vi "GAP_AcquireImagesV3_0.vi"() -> ()   [LabVIEW 2020]
uses:
  <vilib>/vision/driver/IMAQdx.llb/IMAQdx Buffer Number Mode.ctl
  <vilib>/vision/driver/NI_Vision_Acquisition_Software.lvlib
  <vilib>/vision/NI_Vision_Development_Module.lvlib
  <resource>/objmgr/imaqdx.rc
panel:
  out "Histogram":T1(graph)
  in  "Tab Control":enum32{"Acquisition"}(tab)
  in  "Camera Name":refnum<k21> caption="IMAQdx Session"
  out "Original Image":T2(plugin-control)
  out "Grayscale Image":T2(plugin-control)
  out "Acquired imgs":u32
  out "Frame rate":dbl
  in  "Overwrite Mode":u16(ring) items=["Get Oldest"=0, "Fail"=2, "Get Newest"=3]
  in  "Percent of Images Reserved by Driver":dbl=50.0
  out "Line profile data":T3 {"Minimum grayscale value" format="%.2f"; "Std. dev. of pixels values [ % ]" format="%.2f"; "Mean value of pixels values" format="%.2f"; "Maximum grayscale value" format="%.2f"}
  out "Line Profile":cluster{"x0":sgl, "dx":sgl, "Pixels Line":sgl[]}(graph)
  in  "Start acquisition":bool
  in  "Stop image acquisition":bool
  in  "Save image":bool
  in  "Stop program":bool
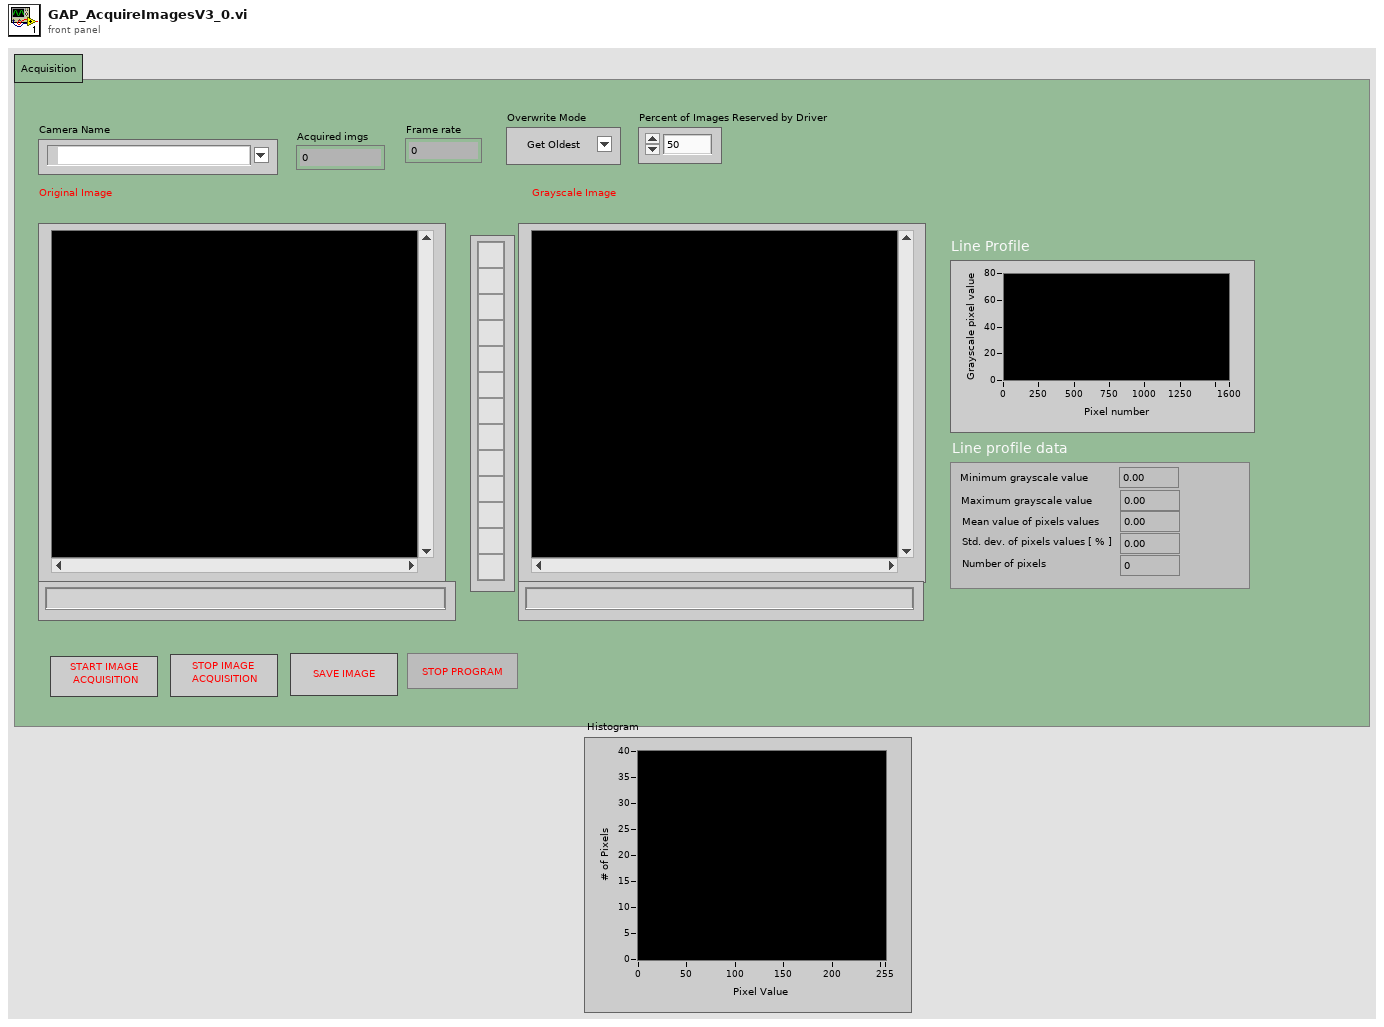
[diagram p1: front panel]
types:
  T1 = cluster{"Starting Value":sgl, "Incremental Value":sgl, "Histogram":u32[]}
  T2 = typedef "IMAQ Image.ctl" = refnum<image>
  T3 = cluster{"Minimum grayscale value":sgl, " Maximum grayscale value":sgl, "Mean value of pixels values":sgl, "Std. dev. of pixels values [ % ]":sgl, "Number of pixels":i32}
  T4 = typedef "NI_Vision_Acquisition_Software.lvlib/IMAQdx Buffer Number Mode.ctl" = enum32{"Next", "Last", "Buffer Number", "Every", "Last New"}
  T5 = typedef "Image Type" = u32
  T6 = typedef "IMAQdx.ctl" = refnum<k21>
  T7 = cluster{"Min":sgl, "Max":sgl, "Mean":sgl, "Std Dev":sgl, "Count":i32}
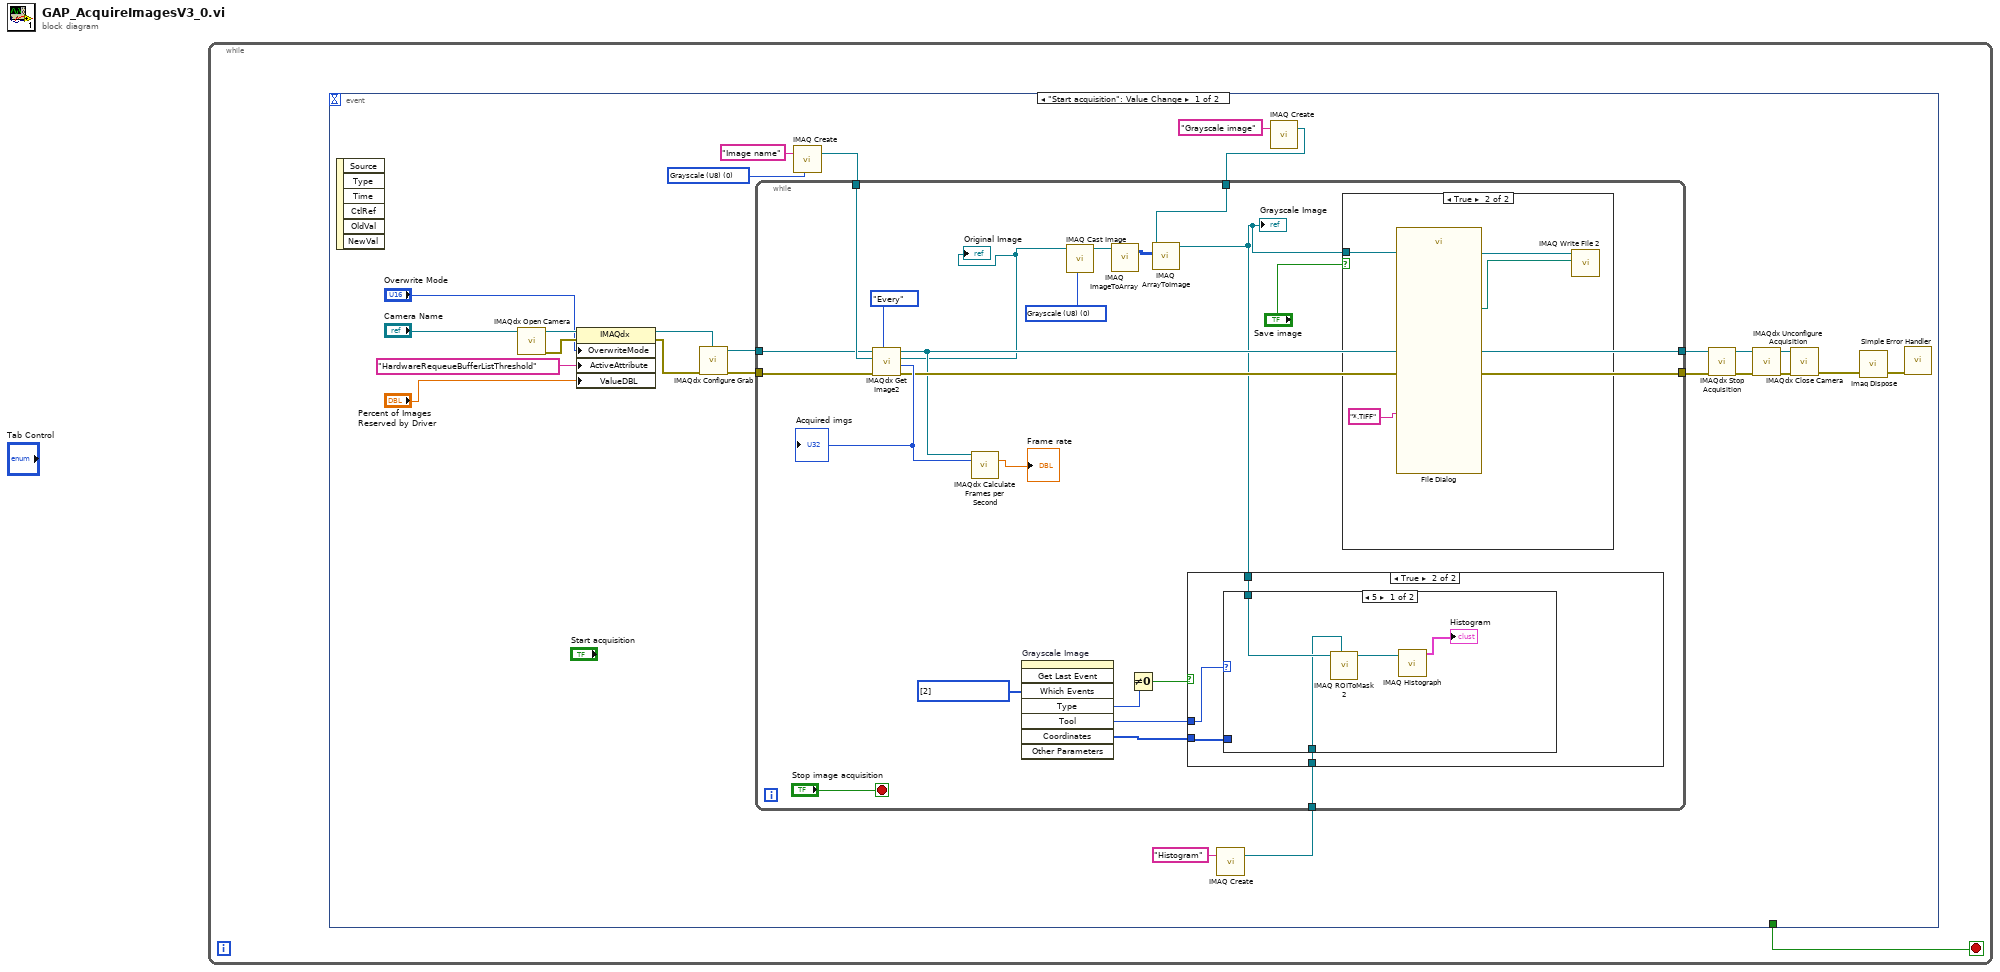
[diagram p0: block diagram]
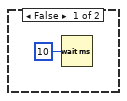
[diagram p3: hidden frame]
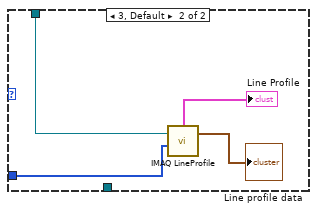
[diagram p4: hidden frame]
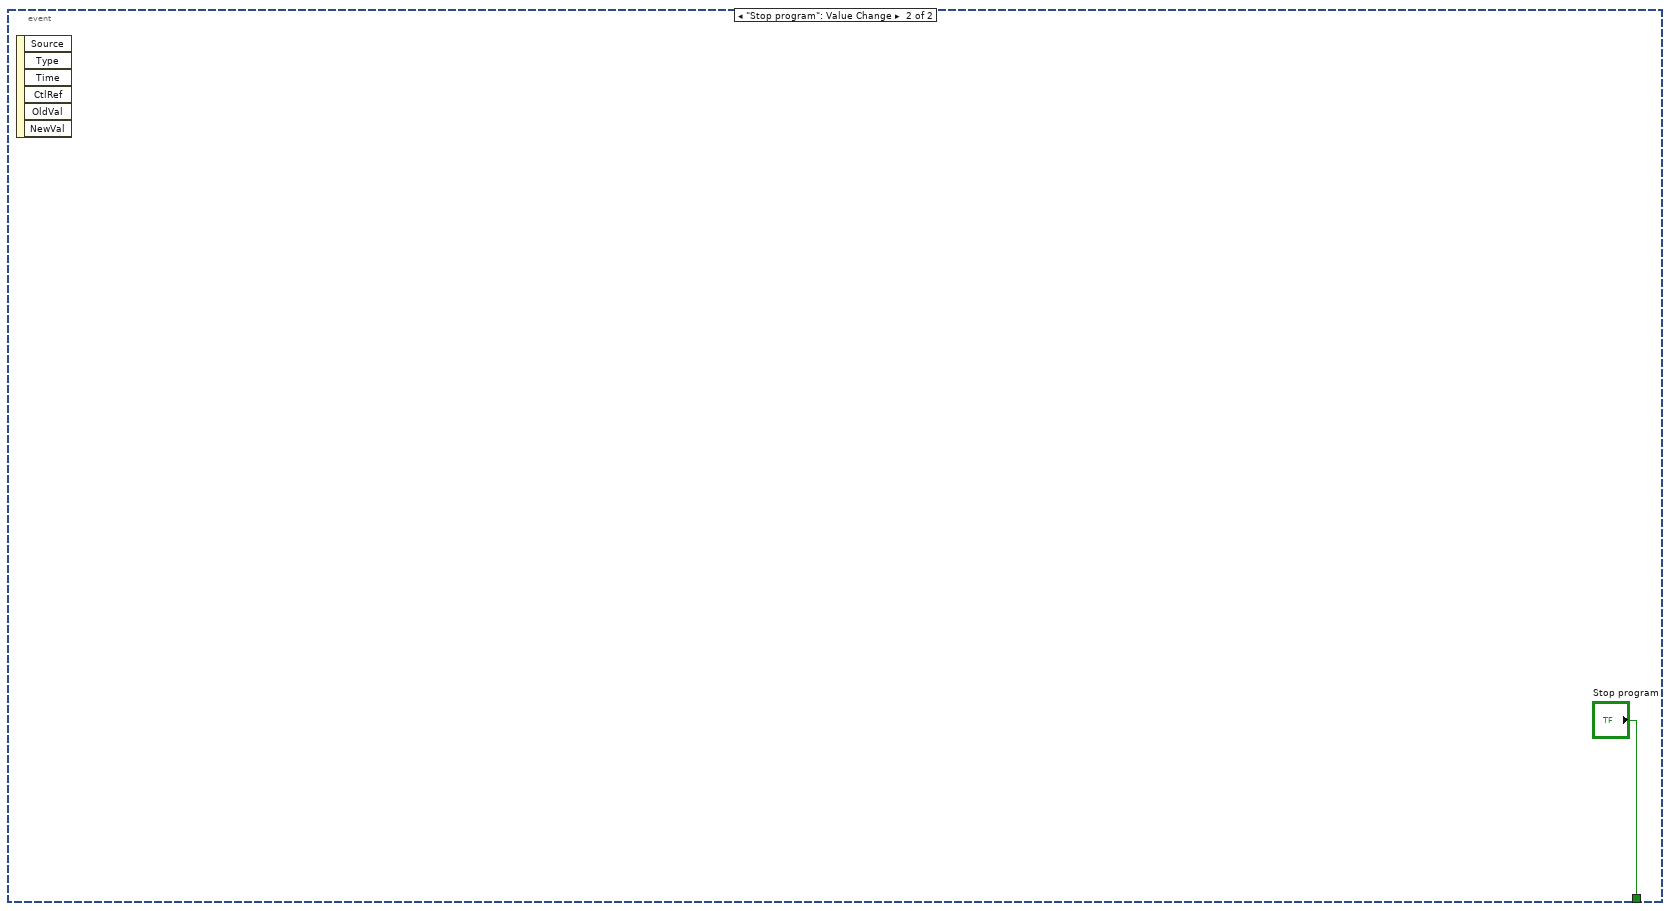
[diagram p5: hidden frame]
diagram:
  n1 = while {
    stop <- w1 stop-if-true
    n2 = event shown="[0] \"Start acquisition\": Value Change" {
      selector: _ -> [_ _]
      dyn-events: _ -> [_ _]
      timeout: _ -> [_ _]
      tunnel: [_ "Stop program"] -> w1
      event "Start acquisition": Value Change {
        w4 = T5 0 items=["Grayscale (U8)", "Grayscale (I16)", "Grayscale (SGL)", "Complex (CSG)", "RGB (U32)", "HSL (U32)", "RGB (U64)", "Grayscale (U16)"] ("Image Type")
        n3 = event-data() -> ()  [unwired: 1 in, 6 out]
        n4 = call <vilib>:"IMAQdx Open Camera.vi"("Session In"="Camera Name") -> ("error out"=w23:errorcluster, "Session Out"=w24:T6)  [unwired: 2 in, 7 out]
        n5 = property class="IMAQdx"(reference=w24, error in=w23, "OverwriteMode"="Overwrite Mode", "ActiveAttribute"="HardwareRequeueBufferListThreshold", "ValueDBL"="Percent of Images Reserved by Driver") -> (reference out=w19:T6, error out=w20:errorcluster)
        n6 = call <vilib>:"IMAQdx Configure Grab.vi"("error in"=w20, "Session In"=w19) -> ("error out"=w17:errorcluster, "Session Out"=w18:T6)  [unwired: 8 in]
        n7 = call "IMAQ Create"("Image Name"="Image name", "Image Type"=w4) -> ("New Image"=w15:T2)  [unwired: 2 in, 2 out]
        n8 = call "IMAQ Create"("Image Name"="Histogram") -> ("New Image"=w2:T2)  [unwired: 3 in, 2 out]
        n9 = call "IMAQ Create"("Image Name"="Grayscale image") -> ("New Image"=w5:T2)  [unwired: 3 in, 2 out]
        n10 = while {
          tunnel: w15 -> [w47]
          tunnel: w18 -> [w45]
          tunnel: w17 -> [w44]
          tunnel: [w43] -> w8
          tunnel: [w42] -> w7
          tunnel: w5 -> [w32]
          tunnel: w2 -> [w27]
          stop <- "Stop image acquisition" stop-if-true
          w35 = T5 0 items=["Grayscale (U8)", "Grayscale (I16)", "Grayscale (SGL)", "Complex (CSG)", "RGB (U32)", "HSL (U32)", "RGB (U64)", "Grayscale (U16)"] ("Image Type")
          w41 = i32[] [2] items=["No Event"=0, "Click Event"=1, "Draw Event"=2, "Size Event"=4, "Scroll Event"=5, "Double Click Event"=8] ("Which Events")
          n11 = call <vilib>:"IMAQdx Get Image2.vi"("Buffer Number Mode (Next)"=IMAQdx_Buffer_Number_Mode."Every", "error in"=w44, "Image In"=w47, "Session In"=w45) -> ("error out"=w43:errorcluster, "Buffer Number Out"=w48:u32, "Image Out"=w31:T2, "Session Out"=w42:T6)  [unwired: 4 in]
          "Acquired imgs" <- w48
          "Original Image" <- w31
          n12 = call <vilib>:"IMAQdx Calculate Frames per Second.vi"("Session In"=w42, "Buffer Number"=w48) -> ("Acquired Frames per Second"=→"Frame rate":dbl)  [unwired: 7 in, 6 out]
          n13 = invoke on="Grayscale Image" class="ImageControl" method="Get Last Event"("Which Events"=w41) -> ("Type"=w40:i32, "Tool"=w28:i32, "Coordinates"=w38:i32[])  [unwired: 7 in, 5 out]
          n14 = call "IMAQ Cast Image"("Image Type"=w35, "Image Src"=w31) -> ("Image Dst Out"=w34:T2)  [unwired: 4 in, 5 out]
          n15 = call "IMAQ ImageToArray"("Image"=w34) -> ("Image Pixels (U8)"=w33:u8[][])  [unwired: 3 in, 4 out]
          n16 = Not Equal To 0?(x=w40) -> (x != 0?=w39:bool)
          n17 = call "IMAQ ArrayToImage"("Image Pixels (U8)"=w33, "Image"=w32) -> ("Image Out"=w30:T2)  [unwired: 8 in, 1 out]
          "Grayscale Image" <- w30
          n18 = case shown="True" w39 {
            tunnel: w38 -> [_ w56]
            tunnel: w30 -> [_ w55]
            tunnel: w28 -> [_ w54]
            tunnel: w27 -> [_ w53]
            frame False {
              n19 = Wait (ms)(milliseconds to wait=u32 10) -> ()  [unwired: 1 out]
            }
            frame True {
              n20 = case shown="5" w54 {
                tunnel: w56 -> [_ w64]
                tunnel: w55 -> [w60 w63]
                tunnel: w53 -> [w58 _]
                frame 5 {
                  n21 = call "IMAQ ROIToMask 2"("Image Model"=w58, "Image"=w60) -> ("Image Out"=w59:T2)  [unwired: 7 in, 2 out]
                  n22 = call "IMAQ Histograph"("Image"=w59) -> ("Histogram Graph"=→"Histogram":T1)  [unwired: 7 in, 3 out]
                }
                frame 3, Default {
                  n23 = call "IMAQ LineProfile"("Line Coordinates"=w64, "Image"=w63) -> ("Line Graph"=→"Line Profile":cluster{"x0":sgl, "dx":sgl, "Pixels Line":sgl[]}, "Line Information"=→"Line profile data":T7)  [unwired: 3 in, 2 out]
                }
              }
            }
          }
          n24 = case shown="True" "Save image" {
            tunnel: w30 -> [_ w51]
            frame False {
            }
            frame True {
              n25 = call "File Dialog"("pattern (all files)"="*.TIFF" ("pattern label")) -> ("selected path"=w50:path)  [unwired: 11 in, 3 out]
              n26 = call-poly "IMAQ Write File 2"("File Path"=w50, "Image"=w51) -> ()  [unwired: 8 in, 2 out]
            }
          }
        }
        n27 = call <vilib>:"IMAQdx Stop Acquisition.vi"("error in"=w8, "Session In"=w7) -> ("error out"=w10:errorcluster, "Session Out"=w11:T6)  [unwired: 8 out]
        n28 = call <vilib>:"IMAQdx Unconfigure Acquisition.vi"("error in"=w10, "Session In"=w11) -> ("error out"=w12:errorcluster, "Session Out"=w13:T6)  [unwired: 8 out]
        n29 = call <vilib>:"IMAQdx Close Camera.vi"("error in"=w12, "Session In"=w13) -> ("error out"=w9:errorcluster)  [unwired: 9 out]
        n30 = call "Imaq Dispose"("error in (no error)"=w9) -> ("error out"=w14:errorcluster)  [unwired: 5 in]
        n31 = call <vilib>:"Simple Error Handler.vi"("error in (no error)"=w14) -> ()  [unwired: 4 in, 5 out]
      }
      event "Stop program": Value Change {
        n32 = event-data() -> ()  [unwired: 1 in, 6 out]
      }
    }
  }
